vi "shutdown stream.vi"(11 "stream session":refnum<data-value>) -> (0 "error out":errorcluster)   [LabVIEW 2020, in "nominal core steps.lvlib"]
doc: "Closes the stream connection."
uses:
  nominal core steps.lvlib
  stream session.ctl
  <vilib>/Nominal/Nominal IO Client/submodules/nominal-streaming-labview-ffi/lv_src/Stream/Stream.lvclass
  channel uid.ctl
  <vilib>/Nominal/Nominal IO Client/submodules/nominal-streaming-labview-ffi/lv_src/Channel/Channel.lvclass
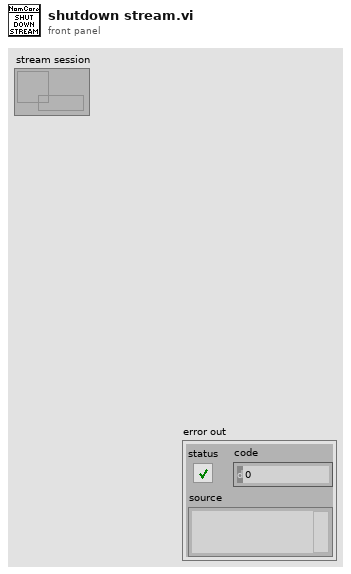
[diagram p1: front panel]
types:
  T1 = typedef "nominal core steps.lvlib/stream session.ctl" = cluster{"Stream":refnum<class "Stream.lvclass">, "channel cache":map{T2, refnum<class "Channel.lvclass">}}
  T2 = typedef "nominal core steps.lvlib/channel uid.ctl" = cluster{"channel name":string, "tags":map{string, string}}
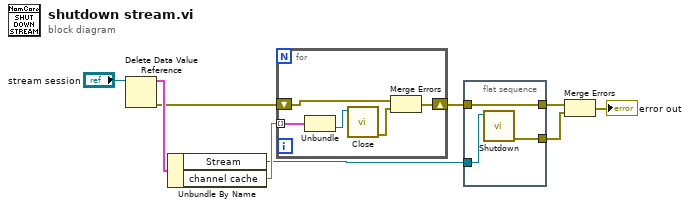
[diagram p0: block diagram]
diagram:
  n1 = Delete Data Value Reference(data value reference="stream session") -> (data value=w7:T1, error out=w5:errorcluster)  [unwired: 1 in]
  n2 = Unbundle By Name(w7) -> ("Stream"=w3:refnum<class "Stream.lvclass">, "channel cache"=w6:map{T2, refnum<class "Channel.lvclass">})
  n3 = for {
    tunnel: w6 -> [w14] mode=indexing
    shift-right: [w12] -> w1
    shift-left: w5 -> [w11]
    n4 = Unbundle(w14) -> ("Channel"=w13:refnum<class "Channel.lvclass">)  [unwired: 1 out]
    n5 = call <vilib>:"Close.vi"("Channel in"=w13) -> ("error out"=w10:errorcluster)  [unwired: 10 in]
    n6 = Merge Errors(w11, w10) -> (w12:errorcluster)
  }
  n7 = flat-sequence {
    tunnel: [w17] -> w4
    tunnel: w3 -> [w16]
    tunnel: [w15] -> w2
    tunnel: w1 -> [w15]
    frame #0 {
      n8 = call <vilib>:"Shutdown.vi"("Nominal Streaming in"=w16) -> ("error out"=w17:errorcluster)  [unwired: 9 in, 1 out]
    }
  }
  n9 = Merge Errors(w2, w4) -> (→"error out":errorcluster)
